vi "Check Tool Arguments.vi"(8 "error in":errorcluster, 9 "server id":i32, 10 "message json":string, 11 "response":string) -> (0 "error out":errorcluster, 3 "response out":string)   [LabVIEW 2020, in "MCP Server.lvlib"]
doc: "Checks that a tools/call request gives every required input of the tool. A required input is one that is set to Required on the connector pane of the tool VI (tools/list lists it in inputSchema.required).\n\nIf the tool is registered, arguments is missing or a JSON object, and one or more required inputs are not in it:\n- error out is LabVIEW error 402841 (the code JSONtext uses for a missing item) with the text Missing required argument(s): followed by the names. Wired to Call VI.vi, this keeps the tool from running.\n- response out is a tools/call result with isError true and that text as its only content item, with the id of the request. Since MCP 2025-11-25 an input validation error is a tool execution error, not a protocol error, so that the model can correct the call.\nOtherwise error out is error in and response out is response.\n\nArguments that the tool does not have are not checked here. tool call.vi calls this VI twice: before Call VI.vi on the error wire, and at the end on the response wire. Check Prompt Arguments.vi does the same for prompts/get, where a missing argument stays a JSON-RPC error."
uses:
  MCP Server.lvlib
  f80f44e1-a1a0-4e1a-a850-eb665eef4700.vi
  32a0083b-af32-4388-8c12-f204ff2875b6.vi
  88c2f0e1-691f-44ea-a9e3-4910211054f9.vi
  <vilib>/JDP Science/JSONtext/Next JSON Value.vi
  <vilib>/JDP Science/JSONtext/String Subset.vi
  <vilib>/JDP Science/JSONtext/Parsing/Advance past next JSON Value (inlined COPY).vi
  <vilib>/JDP Science/JSONtext/Parsing/Advance past whitespace.vi
  <vilib>/JDP Science/JSONtext/Parsing/Advance past String.vi
  <vilib>/JDP Science/JSONtext/Parsing/Advance past Number.vi
  <vilib>/JDP Science/JSONtext/Parsing/Advance past Line Ending.vi
  <vilib>/JDP Science/JSONtext/Parsing/Parse Full Path or Item Name.vi
  <vilib>/JDP Science/JSONtext/Parsing/Advance past Array.vi
  <vilib>/JDP Science/JSONtext/Parsing/Advance past Object.vi
  <vilib>/JDP Science/JSONtext/support/Error Cluster From Code.vi
  <vilib>/JDP Science/JSONtext/Offset/Find Item Locations by Path.vi
  <vilib>/JDP Science/JSONtext/JSON text to Variant.vi
  <vilib>/JDP Science/JSONtext/Variant to JSON Text.vi
  <vilib>/JDP Science/JSONtext/LVClass Serializer/JSONtext LVClass Serializer.lvclass
  <vilib>/JDP Science/JSONtext/JSONtext.lvlib
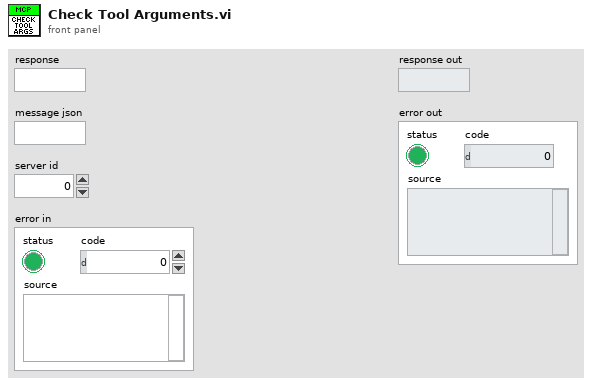
[diagram p1: front panel]
types:
  T1 = typedef "JSONtext.lvlib/JSON Value Type.ctl" = enum16{"Not a JSON Value", "JSON Object", "JSON Array", "String", "Number", "true", "false", "null"}
  T2 = typedef "MCP Server.lvlib/Tool Data.ctl" = cluster{"Name":string, "Description":string, "Ignored":string[], "inputs":T3[], "outputs":T4[], "VI Refnum":refnum<vi>}
  T3 = typedef "MCP Server.lvlib/Input Parameter.ctl" = cluster{"name":string, "type":string, "description":string, "required":bool, "raw name":string, "sub type":string, "array dimension":i32}
  T4 = typedef "MCP Server.lvlib/Output Parameter.ctl" = cluster{"name":string, "description":string, "type":string, "raw name":string}
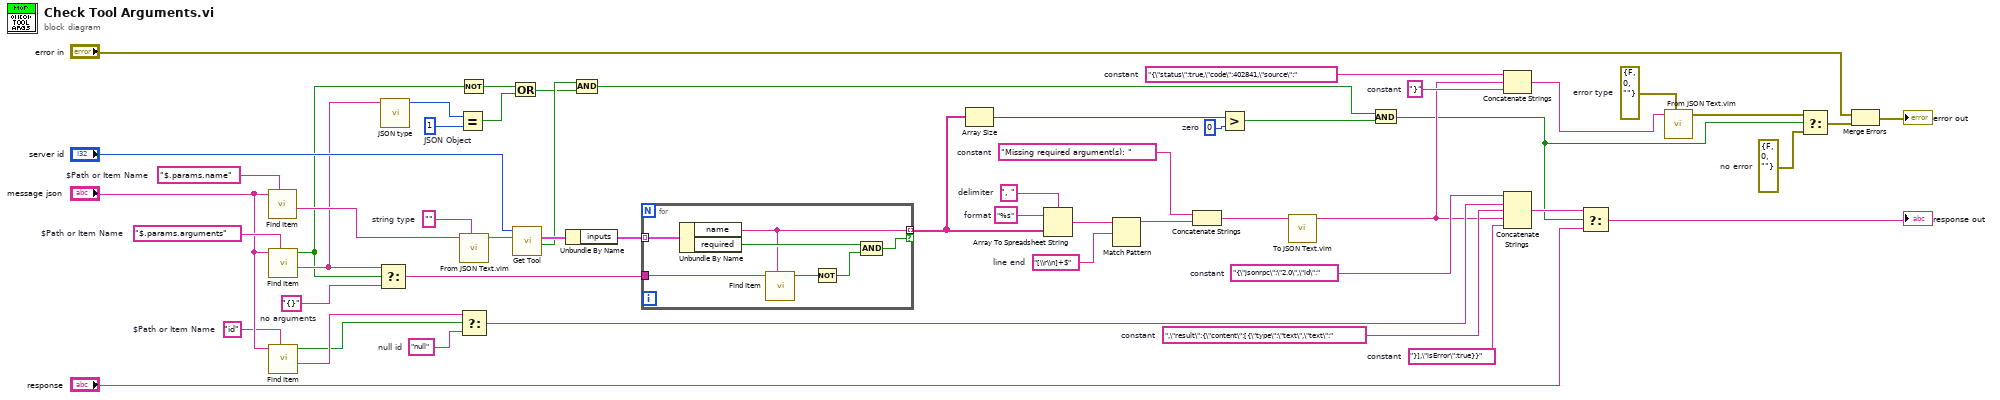
[diagram p0: block diagram]
diagram:
  w6 = "}],\"isError\":true}}"  # constant
  w8 = ",\"result\":{\"content\":[{\"type\":\"text\",\"text\":"  # constant
  w10 = "{\"jsonrpc\":\"2.0\",\"id\":"  # constant
  w11 = "null"  # null id
  w14 = "id"  # $Path or Item Name
  w18 = errorcluster {"status"=FALSE, "code"=0, "source"=""}  # no error
  w20 = errorcluster {"status"=FALSE, "code"=0, "source"=""}  # error type
  w22 = "}"  # constant
  w23 = "{\"status\":true,\"code\":402841,\"source\":"  # constant
  w26 = "Missing required argument(s): "  # constant
  w27 = "[\\r\\n]+$"  # line end
  w29 = ", "  # delimiter
  w31 = "%s"  # format
  w34 = 0  # zero
  w43 = "{}"  # no arguments
  w45 = u16 1  # JSON Object
  w47 = "$.params.arguments"  # $Path or Item Name
  w51 = ""  # string type
  w53 = "$.params.name"  # $Path or Item Name
  n1 = call <vilib>:"Find Item.vi"("$Path or Item Name"=w53, "JSON"="message json") -> ("<JSON>"=w52:string)  [unwired: 6 in, 3 out]
  n2 = call <vilib>:"Find Item.vi"("$Path or Item Name"=w47, "JSON"="message json") -> ("<JSON>"=w44:string, "Found"=w42:bool)  [unwired: 6 in, 2 out]
  n3 = call <vilib>:"Find Item.vi"("$Path or Item Name"=w14, "JSON"="message json") -> ("<JSON>"=w13:string, "Found"=w12:bool)  [unwired: 6 in, 2 out]
  n4 = Select(t=w44, s=w42, f=w43) -> (s? t:f=w36:string)
  n5 = call <vilib>:"JSON type.vi"("JSON"=w44) -> ("JSON Value Type"=w46:T1)  [unwired: 9 in, 1 out]
  n6 = Equal?(x=w46, y=w45) -> (x = y?=w40:bool)
  n7 = Not(x=w42) -> (.not. x?=w41:bool)
  n8 = call "From JSON Text.vim"("Data Type and Default Value"=w51, "JSON"=w52) -> ("Data out"=w49:string)  [unwired: 8 in, 1 out]
  n9 = Select(t=w13, s=w12, f=w11) -> (s? t:f=w9:string)
  n10 = Or(x=w41, y=w40) -> (x .or. y?=w38:bool)
  n11 = call "Get Tool.vi"("Name"=w49, "id in"="server id") -> ("found?"=w39:bool, "Tool Data"=w48:T2)  [unwired: 6 in, 2 out]
  n12 = Unbundle By Name(w48) -> ("inputs"=w37:T3[])
  n13 = And(x=w39, y=w38) -> (x .and. y?=w33:bool)
  n14 = for {
    tunnel: w37 -> [w60] mode=indexing
    tunnel: w36 -> [w59]
    tunnel: [w54] -> w30 mode=indexing if=w55
    n15 = Unbundle By Name(w60) -> ("name"=w54:string, "required"=w57:bool)
    n16 = call <vilib>:"Find Item.vi"("$Path or Item Name"=w54, "JSON"=w59) -> ("Found"=w58:bool)  [unwired: 6 in, 3 out]
    n17 = Not(x=w58) -> (.not. x?=w56:bool)
    n18 = And(x=w57, y=w56) -> (x .and. y?=w55:bool)
  }
  n19 = Array Size(array=w30) -> (size(s)=w35:i32)
  n20 = Array To Spreadsheet String(delimiter (Tab)=w29, array=w30, 3:w31) -> (spreadsheet string=w28:string)
  n21 = Match Pattern(string=w28, regular expression=w27) -> (before substring=w25:string)  [unwired: 1 in, 3 out]
  n22 = Concatenate Strings(w26, w25) -> (w24:string)
  n23 = Greater?(x=w35, y=w34) -> (0:w32:bool)
  n24 = call "To JSON Text.vim"("Anything"=w24) -> ("<JSON>"=w7:string)  [unwired: 9 in, 1 out]
  n25 = And(x=w33, y=w32) -> (x .and. y?=w4:bool)
  n26 = Concatenate Strings(w23, w7, w22) -> (w21:string)
  n27 = Concatenate Strings(w10, w9, w8, w7, w6) -> (w5:string)
  n28 = Select(t=w5, s=w4, f="response") -> (s? t:f=→"response out":string)
  n29 = call "From JSON Text.vim"("Data Type and Default Value"=w20, "JSON"=w21) -> ("Data out"=w19:errorcluster)  [unwired: 8 in, 1 out]
  n30 = Select(t=w19, s=w4, f=w18) -> (s? t:f=w16:errorcluster)
  n31 = Merge Errors("error in", w16) -> (→"error out":errorcluster)
